vi "Reflection Native Object To String.vi"(8 "error in (no error)":errorcluster, 11 "Object in":refnum<k24>) -> (0 "error out":errorcluster, 2 "Text":string, 3 "Object out":refnum<k24>)   [LabVIEW 2026, in "ToastNotification.lvlib" / "Reflection DotNet.lvlib"]
doc: "Native Object.ToString call. Borrow Object in and copy its string representation into Text. Object out is the same borrowed handle, not an acquired result. Does not close or dispose the object. Null input can produce a native .NET error."
uses:
  Reflection DotNet.lvlib
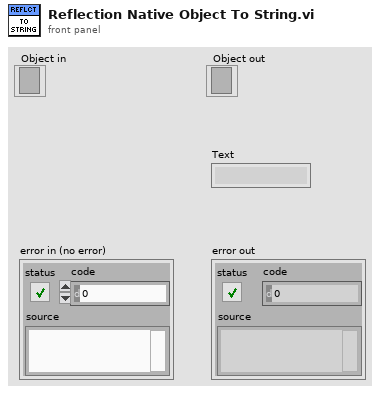
[diagram p1: front panel]
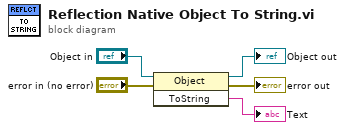
[diagram p0: block diagram]
diagram:
  n1 = invoke class="Object" method="ToString"(reference="Object in", error in="error in (no error)") -> (reference out=→"Object out":refnum<k24>, error out=→"error out":errorcluster, "ToString"=→"Text":string)  [unwired: 1 in]
